vi "clientetcp.vi"() -> ()   [LabVIEW 2017]
panel:
  in  "IP":string="192.168.56.243"
  in  "Port":u16=400
  in  "PARAR":bool
  in  "Izquierda":bool
  in  "Derecha":bool
  in  "VELOCIDAD":dbl(knob) scale=0.0..100.0
  in  "LED2":bool
  in  "LED1":bool
  in  "stop":bool
  # "GIRO"
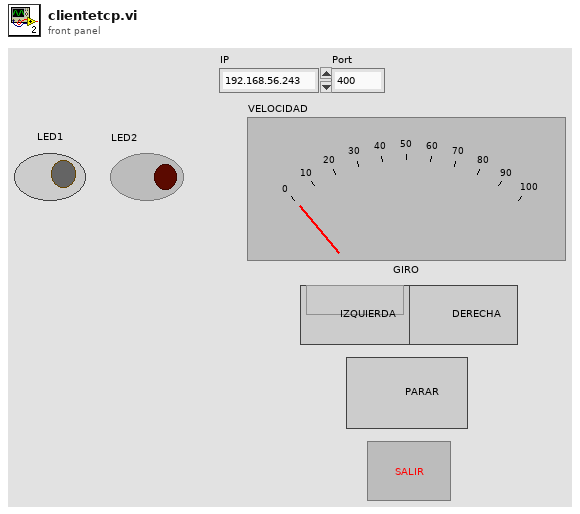
[diagram p1: front panel]
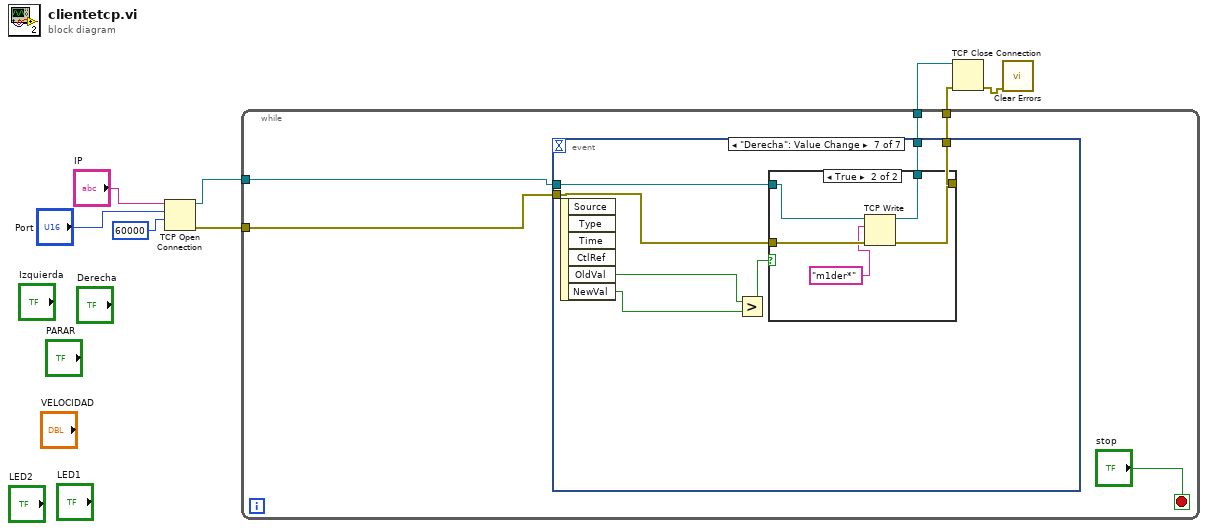
[diagram p0: block diagram]
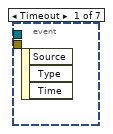
[diagram p2: hidden frame]
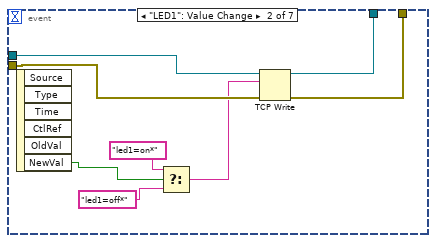
[diagram p3: hidden frame]
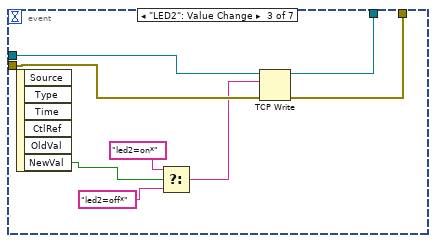
[diagram p4: hidden frame]
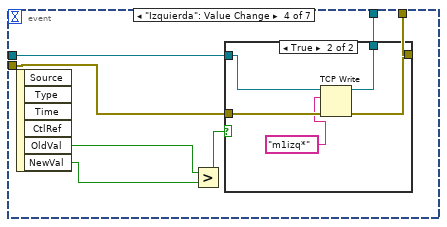
[diagram p5: hidden frame]
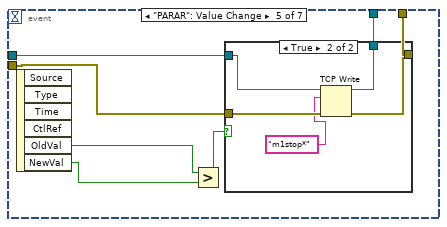
[diagram p7: hidden frame]
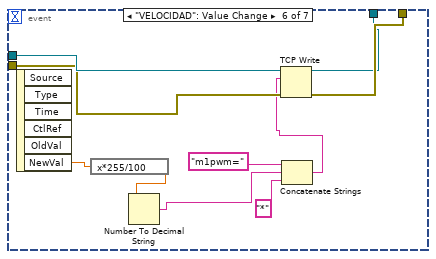
[diagram p9: hidden frame]
diagram:
  n1 = TCP Open Connection(address="IP", remote port or service name="Port", timeout ms (60000)=60000) -> (connection ID=w1:refnum<k5>, error out=w2:errorcluster)  [unwired: 2 in]
  n2 = while {
    tunnel: [w12] -> w8
    tunnel: [w11] -> w7
    tunnel: w2 -> [w10]
    tunnel: w1 -> [w9]
    stop <- "stop" stop-if-true
    n3 = event shown="[6] \"Derecha\": Value Change" {
      selector: _ -> [_ _ _ _ _ _ _]
      dyn-events: _ -> [_ _ _ _ _ _ _]
      timeout: _ -> [_ _ _ _ _ _ _]
      tunnel: w9 -> [_ w21 w29 w36 w48 w63 w70]
      tunnel: w10 -> [_ w20 w28 w35 w47 w62 w69]
      tunnel: [_ w15 w23 w34 w46 w60 w68] -> w12
      tunnel: [_ w14 w22 w33 w45 w61 w67] -> w11
      event Timeout {
        n4 = event-data() -> ()  [unwired: 1 in, 3 out]
      }
      event "LED1": Value Change {
        n5 = event-data() -> ("NewVal"=w19:bool)  [unwired: 1 in, 5 out]
        n6 = Select(t="led1=on*", s=w19, f="led1=off*") -> (s? t:f=w16:string)
        n7 = TCP Write(connection ID=w21, data in=w16, error in (no error)=w20) -> (connection ID out=w15:refnum<k5>, error out=w14:errorcluster)  [unwired: 1 in, 1 out]
      }
      event "LED2": Value Change {
        n8 = event-data() -> ("NewVal"=w27:bool)  [unwired: 1 in, 5 out]
        n9 = Select(t="led2=on*", s=w27, f="led2=off*") -> (s? t:f=w24:string)
        n10 = TCP Write(connection ID=w29, data in=w24, error in (no error)=w28) -> (connection ID out=w23:refnum<k5>, error out=w22:errorcluster)  [unwired: 1 in, 1 out]
      }
      event "Izquierda": Value Change {
        n11 = event-data() -> ("OldVal"=w32:bool, "NewVal"=w31:bool)  [unwired: 1 in, 4 out]
        n12 = Greater?(x=w32, y=w31) -> (0:w30:bool)
        n13 = case shown="True" w30 {
          tunnel: w36 -> [_ w41]
          tunnel: w35 -> [_ w40]
          tunnel: [_ w39] -> w34
          tunnel: [_ w38] -> w33
          frame False {
          }
          frame True {
            n14 = TCP Write(connection ID=w41, data in="m1izq*", error in (no error)=w40) -> (connection ID out=w39:refnum<k5>, error out=w38:errorcluster)  [unwired: 1 in, 1 out]
          }
        }
      }
      event "PARAR": Value Change {
        n15 = event-data() -> ("OldVal"=w44:bool, "NewVal"=w43:bool)  [unwired: 1 in, 4 out]
        n16 = Greater?(x=w44, y=w43) -> (0:w42:bool)
        n17 = case shown="True" w42 {
          tunnel: w48 -> [_ w53]
          tunnel: w47 -> [_ w52]
          tunnel: [_ w51] -> w46
          tunnel: [_ w50] -> w45
          frame False {
          }
          frame True {
            n18 = TCP Write(connection ID=w53, data in="m1stop*", error in (no error)=w52) -> (connection ID out=w51:refnum<k5>, error out=w50:errorcluster)  [unwired: 1 in, 1 out]
          }
        }
      }
      event "VELOCIDAD": Value Change {
        n19 = event-data() -> ("NewVal"=w55:dbl)  [unwired: 1 in, 5 out]
        n20 = expression code="x*255/100"(w55) -> (w54:dbl)
        n21 = Number To Decimal String(number=w54) -> (decimal integer string=w58:string)  [unwired: 1 in]
        n22 = Concatenate Strings("m1pwm=" ("string"), w58, "*" ("string")) -> (w56:string)
        n23 = TCP Write(connection ID=w63, data in=w56, error in (no error)=w62) -> (connection ID out=w60:refnum<k5>, error out=w61:errorcluster)  [unwired: 1 in, 1 out]
      }
      event "Derecha": Value Change {
        n24 = event-data() -> ("OldVal"=w66:bool, "NewVal"=w65:bool)  [unwired: 1 in, 4 out]
        n25 = Greater?(x=w66, y=w65) -> (0:w64:bool)
        n26 = case shown="True" w64 {
          tunnel: w70 -> [_ w75]
          tunnel: w69 -> [_ w74]
          tunnel: [_ w73] -> w68
          tunnel: [_ w72] -> w67
          frame False {
          }
          frame True {
            n27 = TCP Write(connection ID=w75, data in="m1der*", error in (no error)=w74) -> (connection ID out=w73:refnum<k5>, error out=w72:errorcluster)  [unwired: 1 in, 1 out]
          }
        }
      }
    }
  }
  n28 = TCP Close Connection(connection ID=w8, error in (no error)=w7) -> (error out=w6:errorcluster)  [unwired: 1 in, 1 out]
  n29 = call <vilib>:"Clear Errors.vi"("error in (no error)"=w6) -> ()  [unwired: 5 in, 2 out]
